vi "选项卡页面可见.vi"(9 "选项卡可见？":bool, 10 "标题包含字符串":string="7", 11 "选项卡引用":refnum<vi>) -> ()   [LabVIEW 2026, in "UI-无创.lvlib"]
panel:
  in  "错误输出":errorcluster
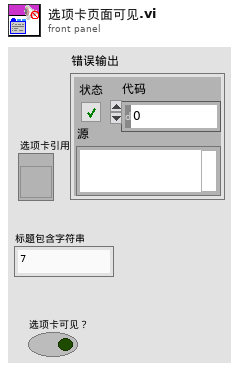
[diagram p1: front panel]
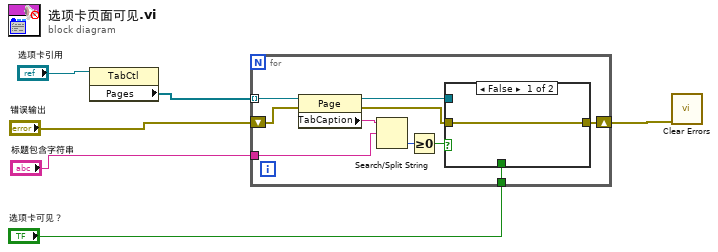
[diagram p0: block diagram]
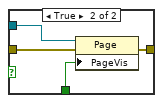
[diagram p2: hidden frame]
diagram:
  n1 = property class="TabCtl"(reference="选项卡引用") -> ("Pages"=w1:refnum<vi>[])  [unwired: 1 in, 2 out]
  n2 = for {
    tunnel: w1 -> [w16] mode=indexing
    tunnel: "标题包含字符串" -> [w11]
    tunnel: "选项卡可见？" -> [w10]
    shift-right: [w9] -> w4
    shift-left: "错误输出" -> [w8]
    n3 = property class="Page"(reference=w16, error in=w8) -> (reference out=w12:refnum<vi>, error out=w7:errorcluster, "TabCaption"=w15:string)
    n4 = Search/Split String(string=w15, search string/char (-)=w11) -> (offset of match=w14:i32)  [unwired: 1 in, 2 out]
    n5 = Greater Or Equal To 0?(x=w14) -> (x >= 0?=w13:bool)
    n6 = case shown="False" w13 {
      tunnel: w12 -> [_ w21]
      tunnel: w10 -> [_ w20]
      tunnel: [w17 w19] -> w9
      tunnel: w7 -> [w17 w18]
      frame False {
      }
      frame True {
        n7 = property class="Page"(reference=w21, error in=w18, "PageVis"=w20) -> (error out=w19:errorcluster)  [unwired: 1 out]
      }
    }
  }
  n8 = call <vilib>:"Clear Errors.vi"("error in (no error)"=w4) -> ()  [unwired: 5 in, 2 out]
